vi "Day Total.vi"(8 "error in":errorcluster, 9 "Now":timestamp, 10 "Day":timestamp, 11 "Entries":T1) -> (0 "error out":errorcluster, 1 "Total Text":string, 2 "Total Seconds":dbl)   [LabVIEW 2026]
doc: "Total time tracked on one local calendar day. Each entry counts only the part of it inside the day, from local midnight of Day to local midnight of the next day (calendar-correct, so a 23- or 25-hour daylight saving day is handled). A running entry (End Time 0) counts up to Now; an entry whose start is after its end or after Now (clock skew) counts 0. Overlapping entries are simply added. Pure arithmetic, no file access, so it can be called on every timer tick.\n\nTotal Text is HH:MM:SS in the style of the TimeCard's Elapsed column: the total is rounded to whole seconds BEFORE it is split, so it never shows :60. Hours are not wrapped at 24 (e.g. 25:03:00). An empty Entries gives 0 and 00:00:00 with no error.\n\nInputs: Entries (e.g. Total Entries from Day Total Entries.vi); Day (any time within the local day); Now (current time); error in (passed through).\nOutputs: Total Seconds; Total Text; error out.\n\nGenerated by: Claude"
uses:
  Storage/Rows/Time Entry List.ctl
  Storage/Rows/Time Entry.ctl
  Utilities/Time Management/Time Management.lvlib
  Utilities/Time Management/ENUM-Inc_Dec.ctl
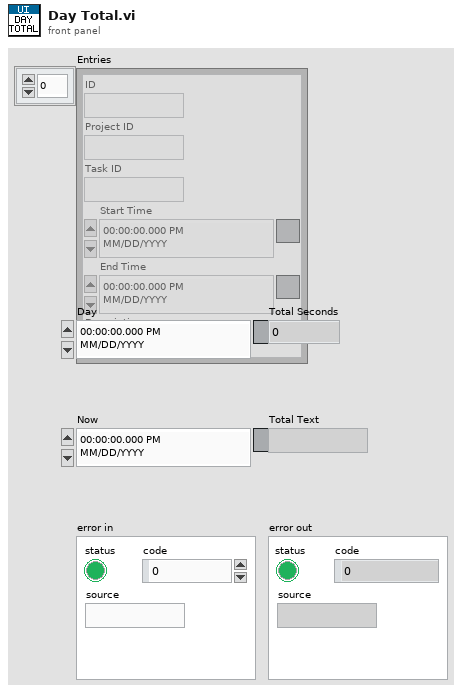
[diagram p1: front panel]
types:
  T1 = typedef "Time Entry List.ctl" = T2[]
  T2 = typedef "Time Entry.ctl" = cluster{"ID":string, "Project ID":string, "Task ID":string, "Start Time":timestamp, "End Time":timestamp, "Description":string}
  T3 = typedef "ENUM-Inc_Dec.ctl" = enum16{"NO CHANGE", "Increment", "Decrement"}
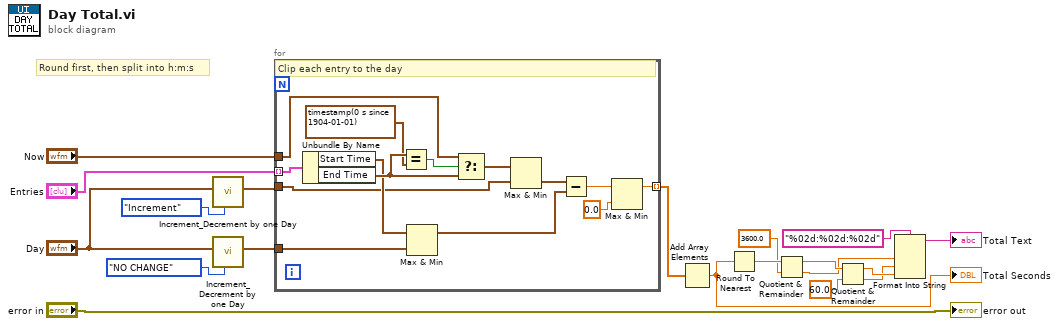
[diagram p0: block diagram]
diagram:
  # "Round first, then split into h:m:s"
  n1 = call "Increment_Decrement by one Day.vi"("Inc/Dec (No Change)"=ENUM-Inc_Dec."Increment" ("Inc/Dec next day"), "Start Day"="Day") -> ("End Day"=w13:timestamp)  [unwired: 8 in, 1 out]
  n2 = call "Increment_Decrement by one Day.vi"("Inc/Dec (No Change)"=ENUM-Inc_Dec."NO CHANGE" ("Inc/Dec same day"), "Start Day"="Day") -> ("End Day"=w12:timestamp)  [unwired: 8 in, 1 out]
  n3 = for {
    tunnel: "Entries" -> [w20] mode=indexing
    tunnel: "Now" -> [w23]
    tunnel: w12 -> [w21]
    tunnel: w13 -> [w22]
    tunnel: [w33] -> w14 mode=indexing
    # "Clip each entry to the day"
    n4 = Unbundle By Name(w20) -> ("Start Time"=w26:timestamp, "End Time"=w27:timestamp)
    n5 = Equal?(x=w27, y=timestamp(0 s since 1904-01-01) ("running End Time")) -> (x = y?=w28:bool)
    n6 = Max & Min(x=w26, y=w21) -> (max(x,y)=w30:timestamp)  [unwired: 1 out]
    n7 = Select(t=w23, s=w28, f=w27) -> (s? t:f=w29:timestamp)
    n8 = Max & Min(x=w29, y=w22) -> (min(x,y)=w31:timestamp)  [unwired: 1 out]
    n9 = Subtract(x=w31, y=w30) -> (x-y=w32:dbl)
    n10 = Max & Min(x=w32, y=0.0 ("no time")) -> (max(x,y)=w33:dbl)  [unwired: 1 out]
  }
  n11 = Add Array Elements(numeric array=w14) -> (sum=w5:dbl)
  "Total Seconds" <- w5
  n12 = Round To Nearest(number=w5) -> (nearest integer value=w15:dbl)
  n13 = Quotient & Remainder(x=w15, y=3600.0 ("seconds per hour")) -> (x-y*floor(x/y)=w17:dbl, floor(x/y)=w16:dbl)
  n14 = Quotient & Remainder(x=w17, y=60.0 ("seconds per minute")) -> (x-y*floor(x/y)=w19:dbl, floor(x/y)=w18:dbl)
  n15 = Format Into String(format string="%02d:%02d:%02d", w16, w18, w19) -> (resulting string=→"Total Text":string)  [unwired: 2 in, 1 out]
  "error out" <- "error in"
